vi "Test Get Pressed Button Index.vi"() -> ()   [LabVIEW 2026]
doc: "Caraya unit test for Get Pressed Button Index.vi, generated by lvai_generate_test.\n\nOne static subVI call per case. Every assertion takes its error in from Define Test rather than from the assertion before it, so a failing case cannot stop a later one - chaining them silently loses cases, measured.\n\nThe error cluster carries the FIRST failure only. Read the JUnit report for all of them."
uses:
  <vilib>/addons/_JKI Toolkits/Caraya/classes/Test/Test.lvclass
  <vilib>/addons/_JKI Toolkits/Caraya/classes/Assert/Assert.lvclass
panel:
  out "error out":errorcluster
  in  "error in":errorcluster
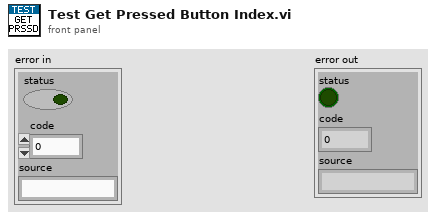
[diagram p1: front panel]
types:
  T1 = cluster{"Func Button":bool, "Func Button 2":bool, "Func Button 3":bool}
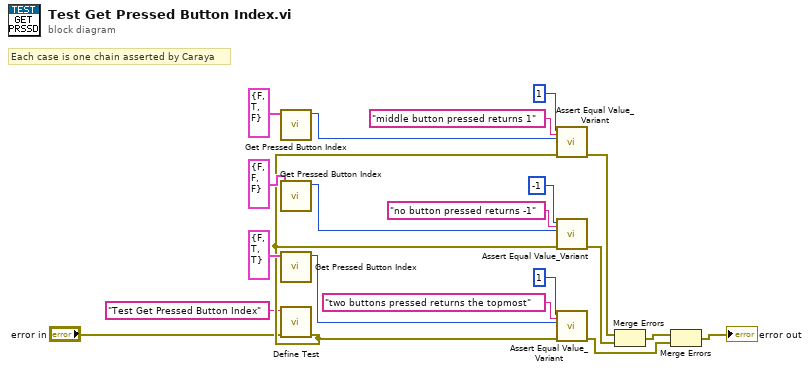
[diagram p0: block diagram]
diagram:
  # "Each case is one chain asserted by Caraya"
  n1 = call "Get Pressed Button Index.vi"("Buttons"=T1 {"Func Button"=FALSE, "Func Button 2"=TRUE, "Func Button 3"=FALSE}) -> ("Button Index"=w5:i32)  [unwired: 9 in, 1 out]
  n2 = call "Get Pressed Button Index.vi"("Buttons"=T1 {"Func Button"=FALSE, "Func Button 2"=FALSE, "Func Button 3"=FALSE}) -> ("Button Index"=w10:i32)  [unwired: 9 in, 1 out]
  n3 = call "Get Pressed Button Index.vi"("Buttons"=T1 {"Func Button"=FALSE, "Func Button 2"=TRUE, "Func Button 3"=TRUE}) -> ("Button Index"=w15:i32)  [unwired: 9 in, 1 out]
  n4 = call <vilib>:"Define Test.vi"("error in (no error)"="error in", "Label (VI Title)"="Test Get Pressed Button Index") -> ("error out"=w3:errorcluster)  [unwired: 8 in, 1 out]
  n5 = call <vilib>:"Assert Equal Value_Variant.vi"("Label"="middle button pressed returns 1", "error in (no error)"=w3, "Actual"=w5, "Expected"=1 ("expected 1")) -> ("error out"=w8:errorcluster)  [unwired: 6 in, 1 out]
  n6 = call <vilib>:"Assert Equal Value_Variant.vi"("Label"="no button pressed returns -1", "error in (no error)"=w3, "Actual"=w10, "Expected"=-1 ("expected 2")) -> ("error out"=w13:errorcluster)  [unwired: 6 in, 1 out]
  n7 = call <vilib>:"Assert Equal Value_Variant.vi"("Label"="two buttons pressed returns the topmost", "error in (no error)"=w3, "Actual"=w15, "Expected"=1 ("expected 3")) -> ("error out"=w18:errorcluster)  [unwired: 6 in, 1 out]
  n8 = Merge Errors(w8, w13) -> (w19:errorcluster)
  n9 = Merge Errors(w19, w18) -> (→"error out":errorcluster)
